vi "FuncVI-FileStripPath.vi"(5 "InstanceRef":T2, 9 "arg list":T1[](array[typedef]) {"num" format="%.2f"}) -> (0 "error out":bool, 3 "result":T1 {"num" format="%.2f"})   [LabVIEW 2021]
doc: "::: CalcExpress Toolkit :::\nCopyright (c) 2000-2026 Konstantin Shifershteyn. All rights reserved."
uses:
  cetypes.llb/CalcExpress Function Argument Info.ctl
  cetypes.llb/CalcExpress Instance RefNum.ctl
panel:
  in  "max arg num":i32=2
  in  "min arg num":i32=1
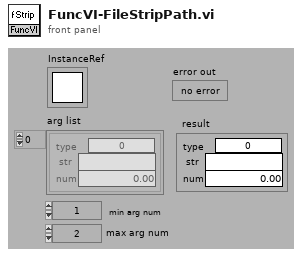
[diagram p1: front panel]
types:
  T1 = typedef "CalcExpress Function Argument Info.ctl" = cluster{"type":u32, "str":string, "num":dbl}
  T2 = typedef "CalcExpress Instance RefNum.ctl" = refnum<k1>
  T3 = cluster{"index":i32, "data type":enum32{"String", "DBL Number", "identifier", "1D Array of DBL", "2D Array of DBL", "CDB Number", "1D Array of CDB", "2D Array of CDB", "1D Array of String", "2D Array of String", "Unknown data type"}, "default num":dbl, "default str":string}[]
  T4 = enum32{"String", "DBL Number", "identifier", "1D Array of DBL", "2D Array of DBL", "CDB Number", "1D Array of CDB", "2D Array of CDB", "1D Array of String", "2D Array of String", "Unknown data type"}
  T5 = cluster{"type: use this constant to specify a predefined type code":enum32{"String", "DBL Number", "identifier", "1D Array of DBL", "2D Array of DBL", "CDB Number", "1D Array of CDB", "2D Array of CDB", "1D Array of String", "2D Array of String", "Unknown data type"}, "name":string, dbl}
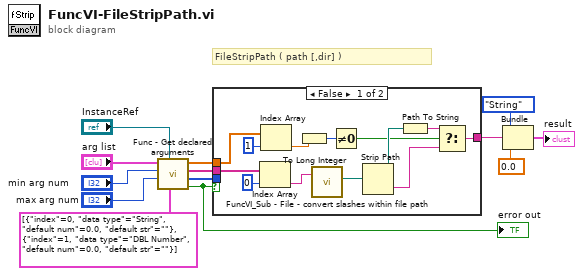
[diagram p0: block diagram]
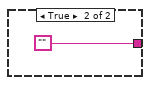
[diagram p2: hidden frame]
diagram:
  # "FileStripPath ( path [,dir] )"
  n1 = call "Func - Get declared arguments.vi"("arg descriptors"=T3 [{"index"=0, "data type"=enum."String", "default num"=0.0, "default str"=""}, {"index"=1, "data type"=enum."DBL Number", "default num"=0.0, "default str"=""}] ("args descriptors"), "InstanceRef"="InstanceRef", "max arg num"="max arg num", "min arg num"="min arg num", "arg list"="arg list") -> ("error out"=w3:bool, "type list"=w7:u32[], "str list"=w9:string[], "num list"=w8:dbl[])  [unwired: 3 in]
  "error out" <- w3
  n2 = case shown="False" w3 {
    tunnel: w9 -> [w21 _]
    tunnel: w8 -> [w24 _]
    tunnel: w7 -> [_ _]
    tunnel: [w17 ""] -> w4
    frame False {
      n3 = Index Array(array=w21, index=0) -> (element=w15:string)
      n4 = Index Array(array=w24, index=1) -> (element=w23:dbl)
      n5 = To Long Integer(number=w23) -> (32bit integer=w22:i32)
      n6 = call "FuncVI_Sub - File - convert slashes within file path.vi"("str: path"=w15) -> ("path out"=w14:path)  [unwired: 3 in, 1 out]
      n7 = Not Equal To 0?(x=w22) -> (x != 0?=w16:bool)
      n8 = Strip Path(path=w14) -> (stripped path=w20:path, name=w19:string)
      n9 = Path To String(path=w20) -> (string=w18:string)
      n10 = Select(t=w18, s=w16, f=w19) -> (s? t:f=w17:string)
    }
    frame True {
    }
  }
  n11 = Bundle("type: use this constant to specify a predefined type code"=T4."String", "name"=w4, 0.0) -> (→"result":T5)  [unwired: 1 in]
